vi "Scratch.vi"() -> ()   [LabVIEW 2026]
panel:
  in  "Set 2":i32
  in  "Set 1":i32
  out "Loop 2-i":i32
  out "Loop 1-i":i32
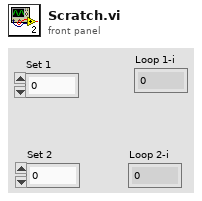
[diagram p1: front panel]
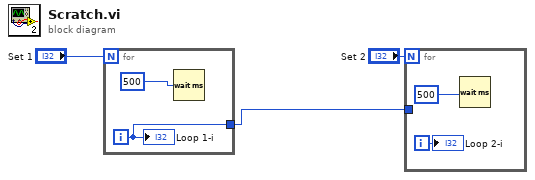
[diagram p0: block diagram]
diagram:
  n1 = for {
    N: "Set 1" -> [_]
    tunnel: [w4] -> w1
    i -> [w4]
    n2 = Wait (ms)(milliseconds to wait=u32 500 ("millisecond timer value")) -> ()  [unwired: 1 out]
    "Loop 1-i" <- w4
  }
  n3 = for {
    N: "Set 2" -> [_]
    tunnel: w1 -> [_]
    i -> [w7]
    n4 = Wait (ms)(milliseconds to wait=u32 500 ("millisecond timer value")) -> ()  [unwired: 1 out]
    "Loop 2-i" <- w7
  }
